vi "Status.vi"(8 "error in (no error)":errorcluster, 11 "Git Updater Module in":refnum<class "Git Updater Module.lvclass">) -> (0 "error out":errorcluster, 2 "Path Statuses":T1[](array[typedef]), 3 "Git Updater Module out":refnum<class "Git Updater Module.lvclass">)   [LabVIEW 2020, in "VolatusGUI.lvlib" / "Git Updater Module.lvclass"]
uses:
  Git Updater Module.lvclass
  Path Status.ctl
  Status.ctl
  <vilib>/Hampel Software Engineering/Git API/Git API/GIT-api.lvclass/GIT-api.ctl
  <vilib>/Hampel Software Engineering/Git API/Git API/GIT-api.lvclass
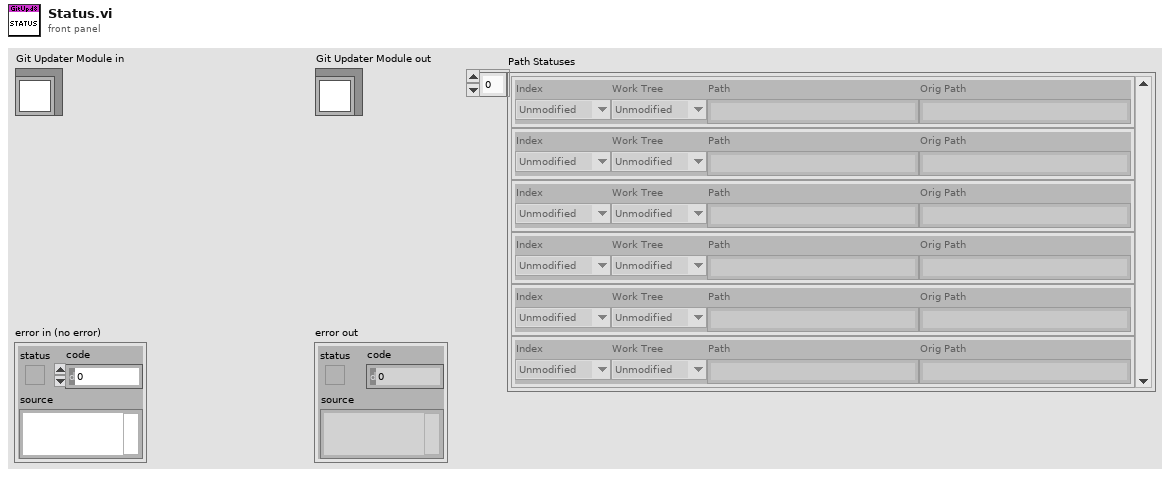
[diagram p1: front panel]
types:
  T1 = typedef "VolatusGUI.lvlib/Git Updater Module.lvclass/Path Status.ctl" = cluster{"Index":T2, "Work Tree":T2, "Path":string, "Orig Path":string}
  T2 = typedef "VolatusGUI.lvlib/Git Updater Module.lvclass/Status.ctl" = enum16{"UNKNOWN", "Unmodified", "Modified", "Added", "Deleted", "Renamed", "Unmerged", "Untracked", "Ignored"}
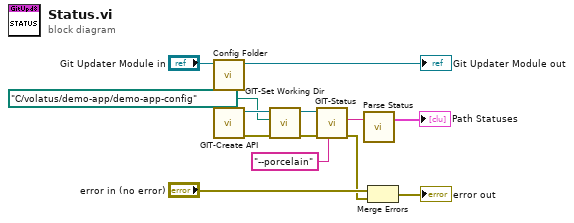
[diagram p0: block diagram]
diagram:
  n1 = call "Config Folder.vi"("Git Updater Module in"="Git Updater Module in") -> ("Git Updater Module out"=→"Git Updater Module out":refnum<class "Git Updater Module.lvclass">)  [unwired: 8 in, 2 out]
  n2 = call <vilib>:"GIT-Create API.vi"() -> ("error out"=w10:errorcluster, "git-api out"=w9:refnum<class "GIT-api.lvclass">)  [unwired: 10 in]
  n3 = call <vilib>:"GIT-Set Working Dir.vi"("error in"=w10, "Working Directory"=path "C:/volatus/demo-app/demo-app-config", "git-api in"=w9) -> ("error out"=w7:errorcluster, "git-api out"=w8:refnum<class "GIT-api.lvclass">)  [unwired: 7 in]
  n4 = call <vilib>:"GIT-Status.vi"("param"="--porcelain", "error in"=w7, "git-api in"=w8) -> ("error out"=w2:errorcluster, "std out"=w5:string)  [unwired: 6 in, 1 out]
  n5 = call "Parse Status.vi"("Status"=w5) -> ("Path Statuses"=→"Path Statuses":T1[])  [unwired: 6 in]
  n6 = Merge Errors("error in (no error)", w2) -> (→"error out":errorcluster)
